vi "Supervisor_Stop_Test.vi"(8 "error in (no error)":errorcluster={"status"=FALSE, "code"=0, "source"="\"\""}, 10 "Stop reason":string, 11 "Active RunContext":string) -> (0 "error out":errorcluster={"status"=FALSE, "code"=0, "source"="\"\""}, 2 "status ok":bool, 3 "Stopping state":string)   [LabVIEW 2026]
doc: "INTENT: Execute operator stop policy. LOGIC: Prevent new normal steps, request cooperative cancellation, revoke leases, run safe shutdown when permitted."
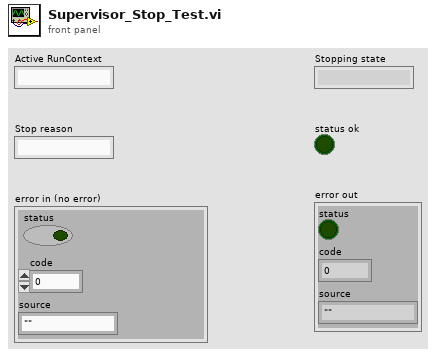
[diagram p1: front panel]
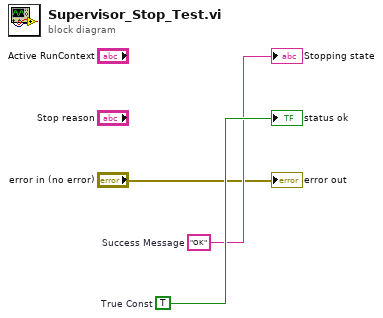
[diagram p0: block diagram]
diagram:
  w3 = TRUE  # True Const
  w2 = "OK"  # Success Message
  "Stopping state" <- w2
  "status ok" <- w3
  "error out" <- "error in (no error)"
